vi "Tester - Array Operations With Bounds Check.vi"() -> ()   [LabVIEW 2026, in "RSysUtils Array.lvlib"]
uses:
  RSysUtils Array.lvlib
  5244ace0-50d1-4baa-b904-a648d470b3f8.vi
  cd8c0fbb-edb6-45d7-9d92-53c8cf8c3ee6.vi
  17da83b0-6c0d-485c-b990-ef888a82906b.vi
  b12056b8-b5af-482c-bafb-d4937d497984.vi
  4db8573a-67e7-4f61-a9c3-5430e5eed4ea.vi
  60ce3f96-f833-447a-a75f-124bd25e91c7.vi
  74036135-4787-4a58-89d4-5e3349ec2971.vi
  19c866c6-3bfb-4b8f-b667-079f2ac444e1.vi
  722d6fb4-19ce-4b55-98ec-8f9e72419cdb.vi
  7834c265-8ff5-4fc6-8135-637b159d0aff.vi
  c15a3146-a81c-44a8-8473-6d10249781a0.vi
  1bc5de83-25e1-46ee-a379-6a5bb9383214.vi
  c7c77501-89cc-4da5-88f4-87423ea7fc09.vi
panel:
  out "1D Array Out 3":string[](array[string])
  out "1D Array Out 2":string[](array[string])
  out "1D Array Out":string[](array[string])
  out "True = Index is in Range 3":bool
  out "True = Index is in Range 2":bool
  out "True = Index is in Range":bool
  # "Tester - Array Operations With Bounds Check"
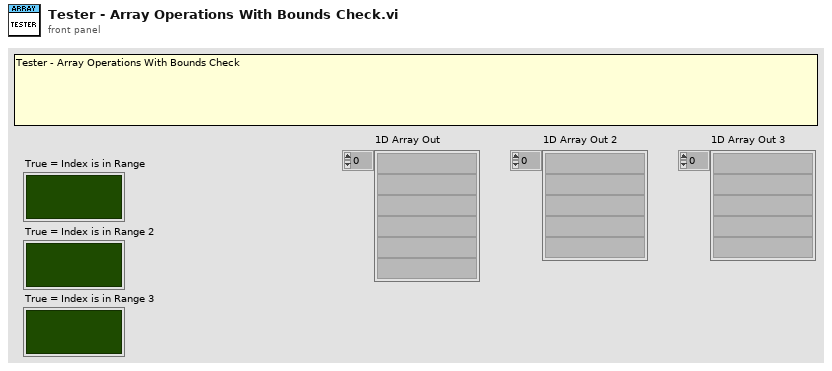
[diagram p1: front panel]
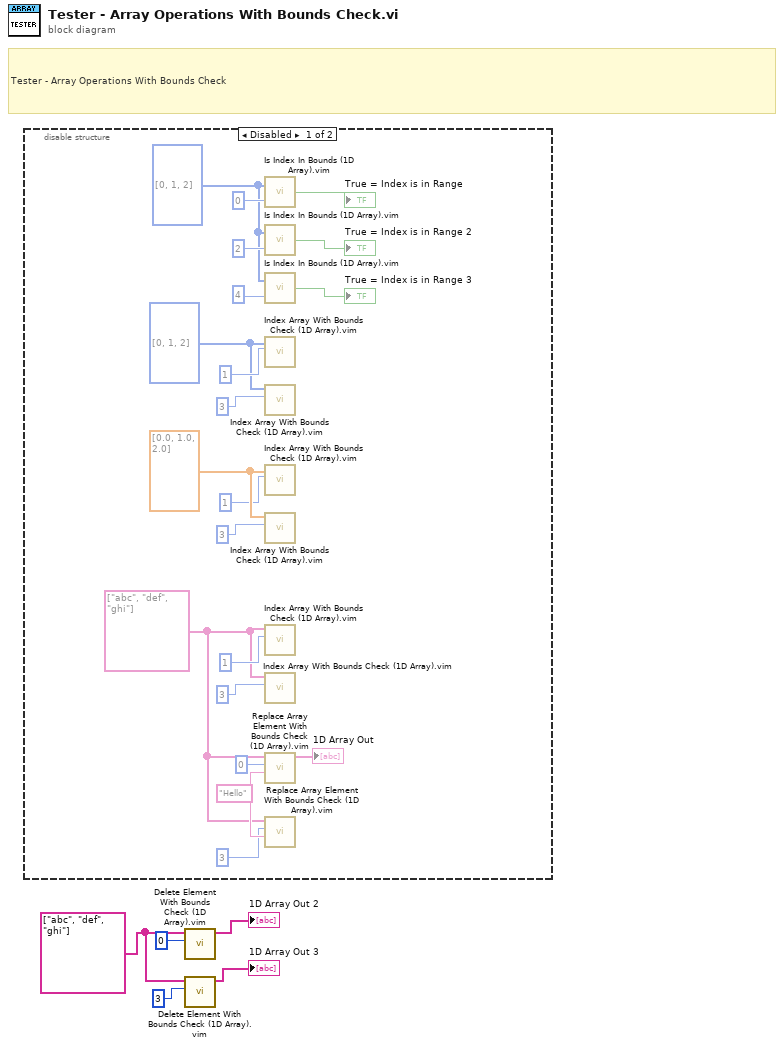
[diagram p0: block diagram]
diagram:
  w3 = string[] ["abc", "def", "ghi"]
  # "Tester - Array Operations With Bounds Check"
  n1 = disable-structure shown="Disabled" {
    frame Disabled {
      w10 = "Hello"
      w6 = string[] ["abc", "def", "ghi"]
      w14 = dbl[] [0.0, 1.0, 2.0]
      w17 = i32[] [0, 1, 2]
      w22 = i32[] [0, 1, 2]
      n2 = call "Is Index In Bounds (1D Array).vim"("Index"=0, "1D Array In"=w22) -> ("Is Index In Bounds?"=→"True = Index is in Range":bool)
      n3 = call "Is Index In Bounds (1D Array).vim"("Index"=2, "1D Array In"=w22) -> ("Is Index In Bounds?"=→"True = Index is in Range 2":bool)
      n4 = call "Is Index In Bounds (1D Array).vim"("Index"=4, "1D Array In"=w22) -> ("Is Index In Bounds?"=→"True = Index is in Range 3":bool)
      n5 = call "Index Array With Bounds Check (1D Array).vim"("Index"=1, "1D Array In"=w17) -> ()  [unwired: 8 in, 2 out]
      n6 = call "Index Array With Bounds Check (1D Array).vim"("Index"=3, "1D Array In"=w17) -> ()  [unwired: 8 in, 2 out]
      n7 = call "Index Array With Bounds Check (1D Array).vim"("Index"=1, "1D Array In"=w14) -> ()  [unwired: 8 in, 2 out]
      n8 = call "Index Array With Bounds Check (1D Array).vim"("Index"=3, "1D Array In"=w14) -> ()  [unwired: 8 in, 2 out]
      n9 = call "Index Array With Bounds Check (1D Array).vim"("Index"=1, "1D Array In"=w6) -> ()  [unwired: 8 in, 2 out]
      n10 = call "Index Array With Bounds Check (1D Array).vim"("Index"=3, "1D Array In"=w6) -> ()  [unwired: 8 in, 2 out]
      n11 = call "Replace Array Element With Bounds Check (1D Array).vim"("New Element"=w10, "Index"=0, "1D Array In"=w6) -> ("1D Array Out"=→"1D Array Out":string[])  [unwired: 7 in, 1 out]
      n12 = call "Replace Array Element With Bounds Check (1D Array).vim"("New Element"=w10, "Index"=3, "1D Array In"=w6) -> ()  [unwired: 7 in, 2 out]
    }
    frame Enabled {
    }
  }
  n13 = call "Delete Element With Bounds Check (1D Array).vim"("Index"=0, "1D Array In"=w3) -> ("1D Array Out"=→"1D Array Out 2":string[])  [unwired: 8 in, 1 out]
  n14 = call "Delete Element With Bounds Check (1D Array).vim"("Index"=3, "1D Array In"=w3) -> ("1D Array Out"=→"1D Array Out 3":string[])  [unwired: 8 in, 1 out]
